vi "Write Type Definition.vi"(8 "error in":errorcluster, 10 "Type Definition":path, 11 "Cluster in":refnum<class "Cluster.lvclass">) -> (0 "error out":errorcluster, 3 "Cluster out":refnum<class "Cluster.lvclass">)   [LabVIEW 2026, in "Cluster.lvclass"]
doc: "Data accessor."
uses:
  Cluster.lvclass
  Cluster.lvclass/Cluster.ctl
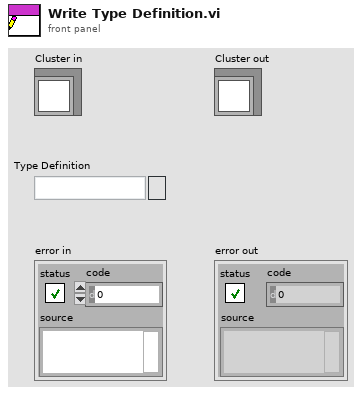
[diagram p1: front panel]
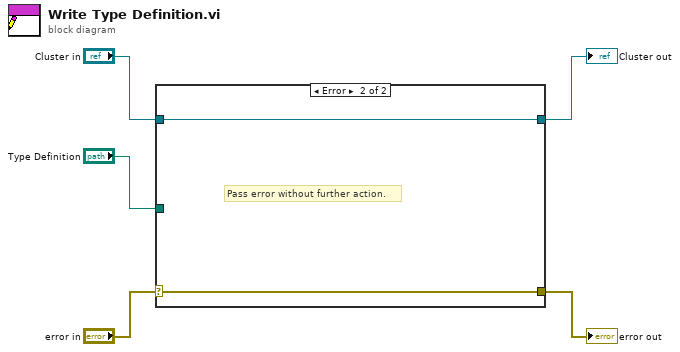
[diagram p0: block diagram]
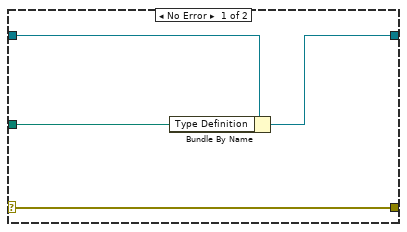
[diagram p2: hidden frame]
diagram:
  n1 = case shown="Error" "error in" {
    selector: "error in" -> [w9 w11]
    tunnel: [w9 w11] -> w4
    tunnel: [w7 w10] -> w2
    tunnel: "Cluster in" -> [w8 w10]
    tunnel: "Type Definition" -> [w6 _]
    frame No Error {
      n2 = Bundle By Name(cluster=w8, "Type Definition"=w6) -> (w7:refnum<class "Cluster.lvclass">)
    }
    frame Error {
      # "Pass error without further action."
    }
  }
  "error out" <- w4
  "Cluster out" <- w2
